vi "VIH HelpGen - HTML - Escape Reserved HTML Characters.vi"(11 "string":string) -> (3 "HTML string":string)   [LabVIEW 2014]
doc: "::: VI Helpeks :::\nCopyright (c) 2000-2026 Konstantin Shifershteyn. All rights reserved."
panel:
  # "VI Helpeks\nCopyright (c) 2012-2026 Konstantin Shifershteyn"
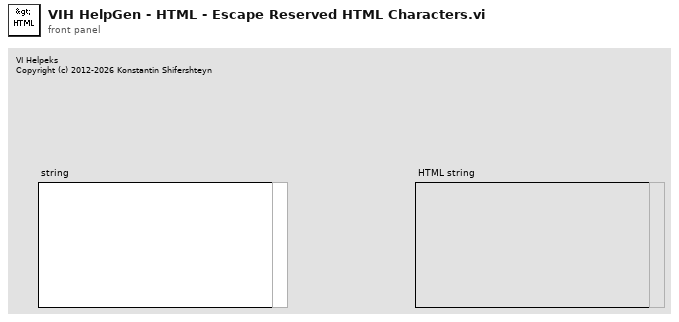
[diagram p1: front panel]
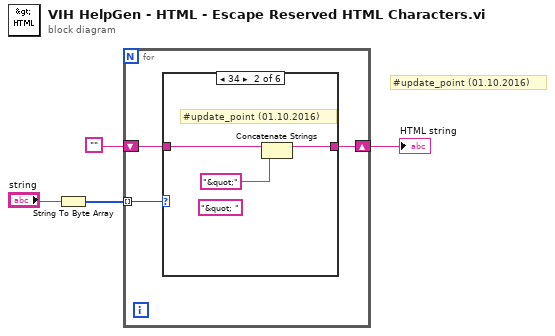
[diagram p0: block diagram]
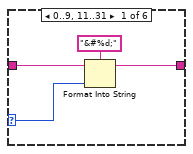
[diagram p2: hidden frame]
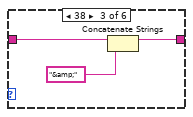
[diagram p3: hidden frame]
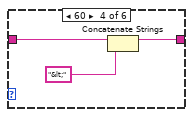
[diagram p4: hidden frame]
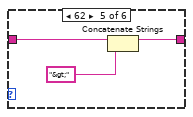
[diagram p5: hidden frame]
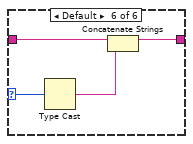
[diagram p6: hidden frame]
diagram:
  # "#update_point (01.10.2016)"
  n1 = String To Byte Array(string="string") -> (unsigned byte array=w3:u8[])
  n2 = for {
    tunnel: w3 -> [w7] mode=indexing
    shift-right: [w5] -> w1
    shift-left: "" -> [w6]
    n3 = case shown="34" w7 {
      selector: w7 -> [w10 _ _ _ _ w25]
      tunnel: w6 -> [w9 w14 w17 w20 w23 w27]
      tunnel: [w8 w13 w16 w19 w22 w26] -> w5
      frame 0..9, 11..31 {
        n4 = Format Into String(format string="&#%d;" ("Format String"), initial string=w9, w10) -> (resulting string=w8:string)  [unwired: 1 in, 1 out]
      }
      frame 34 {
        (unwired) "&quot; "
        # "#update_point (01.10.2016)"
        n5 = Concatenate Strings(w14, "&quot;") -> (w13:string)
      }
      frame 38 {
        n6 = Concatenate Strings(w17, "&amp;") -> (w16:string)
      }
      frame 60 {
        n7 = Concatenate Strings(w20, "&lt;") -> (w19:string)
      }
      frame 62 {
        n8 = Concatenate Strings(w23, "&gt;") -> (w22:string)
      }
      frame Default {
        n9 = Type Cast(x=w25) -> (*(type *) &x=w24:string)  [unwired: 1 in]
        n10 = Concatenate Strings(w27, w24) -> (w26:string)
      }
    }
  }
  "HTML string" <- w1
